vi "1g_v4.vi"() -> ()   [LabVIEW 2017]
uses:
  <vilib>/Instr/_visa.llb/VISA Configure Serial Port (Instr).vi
panel:
  in  "stop":bool
  out "Spectrometer Information":string
  out "Spectrometer Name":string
  in  "Integration Time 100 tp 250 milliseconds":dbl=100.0 min=100.0 max=500.0 step=50.0
  out "XY Graph":cluster{dbl[], u16[]}(graph)
  out "VISA resource name out":refnum<visa-resource-name>
  in  "VISA resource name":refnum<visa-resource-name>="COM3" caption="Serial COM port"
  # "REAL TIME FIBER OPTIC TEMPERATURE MONITORING SYSTEM"
  # "Partially working code"
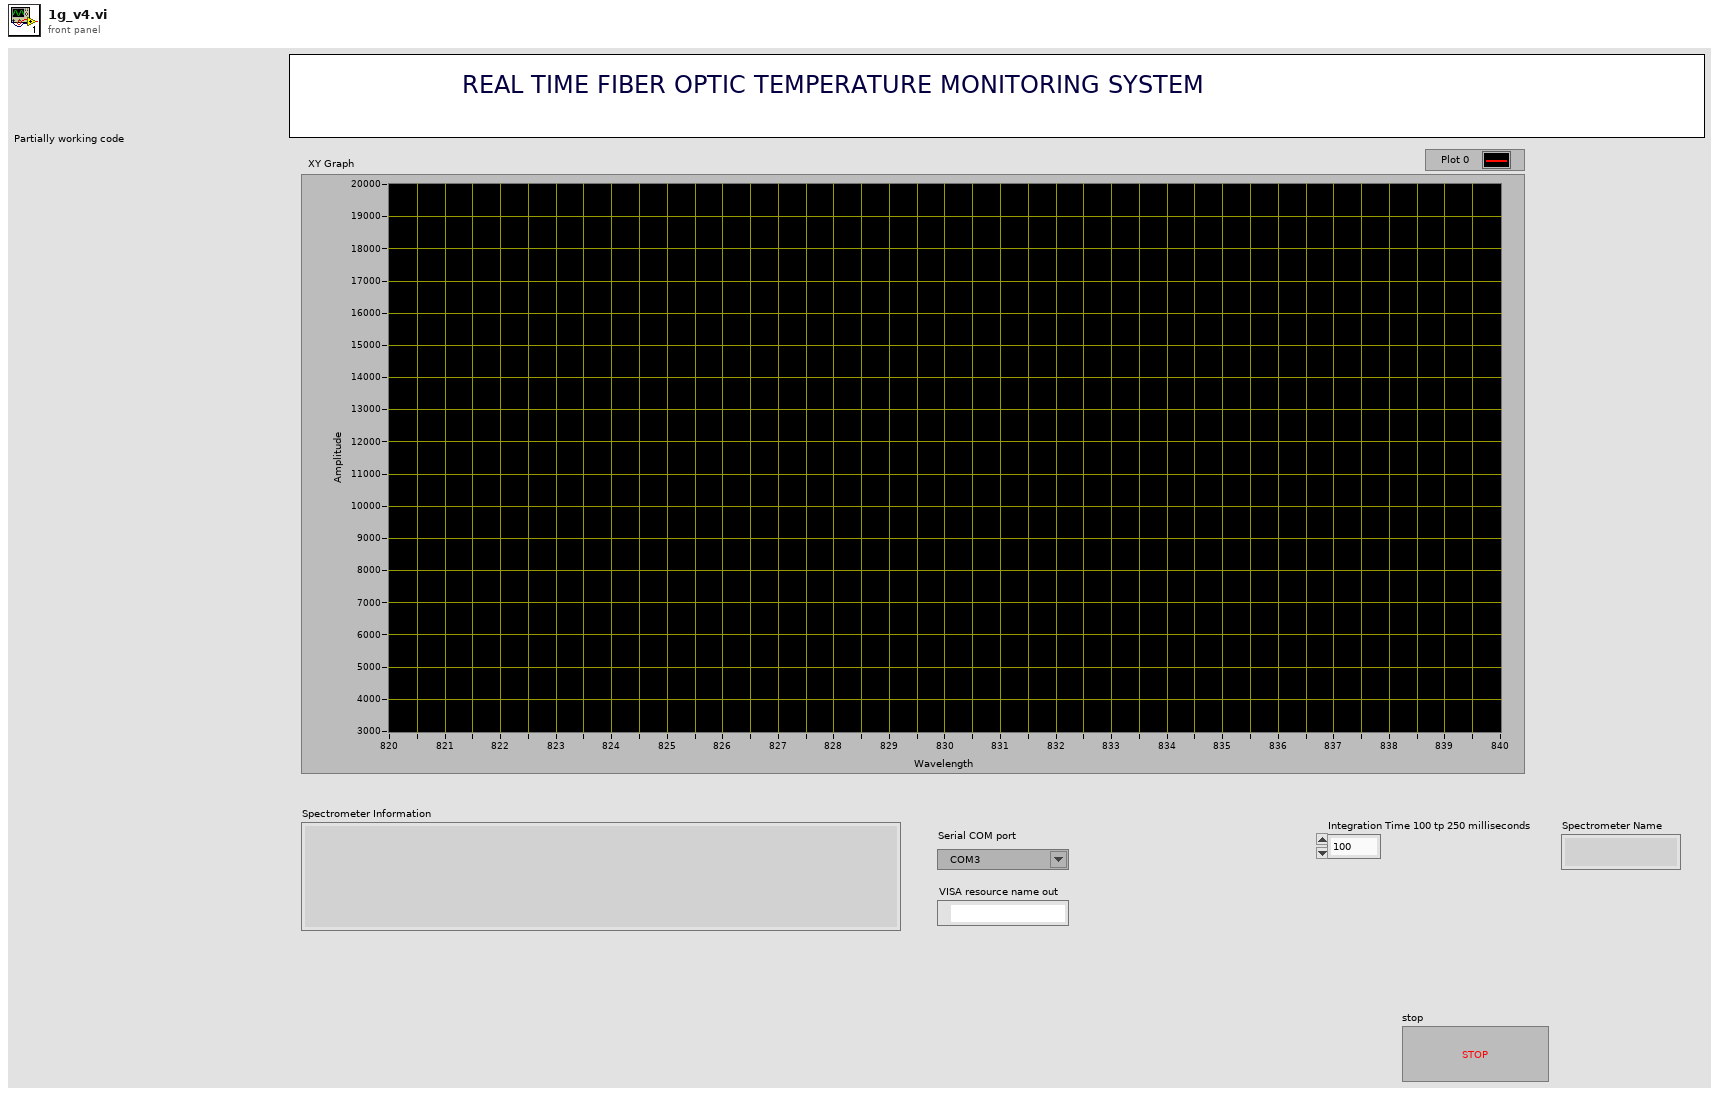
[diagram p1: front panel]
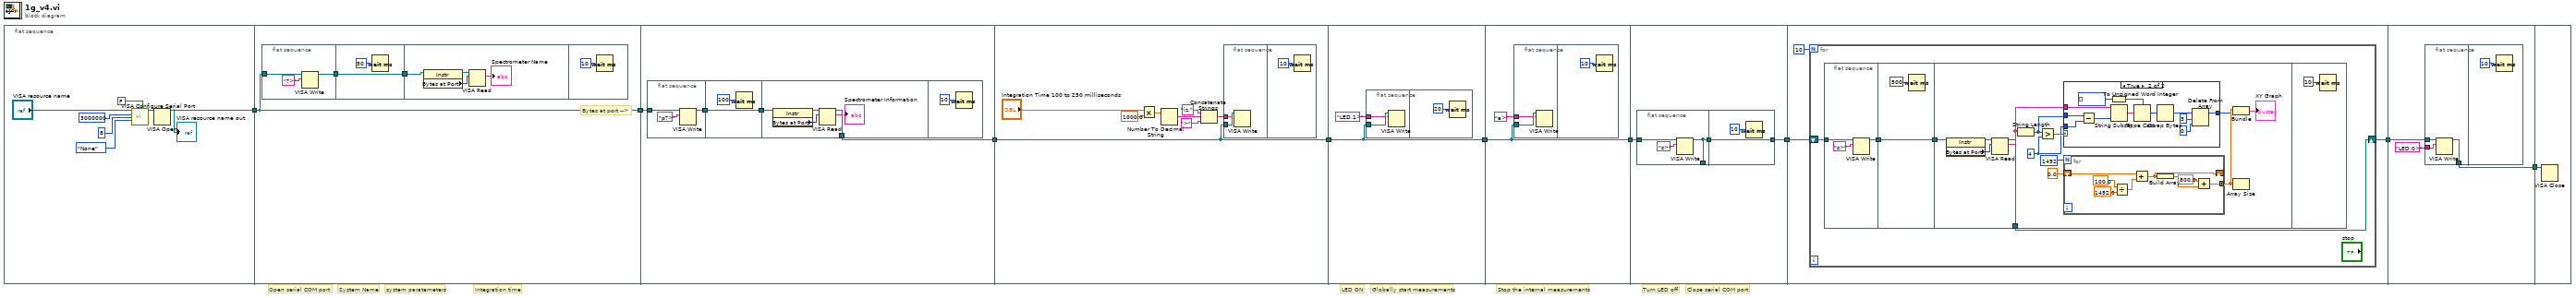
[diagram p0: block diagram]
diagram:
  # "Globally start measurements"
  # "LED ON"
  # "System Name"
  # "Integration time"
  # "system paratemeters"
  # "Close serial COM port"
  # "Turn LED off"
  # "Stop the internal measurements"
  # "Open serial COM port"
  n1 = flat-sequence {
    tunnel: [w10] -> w3
    tunnel: [w17] -> w9
    tunnel: w3 -> [w17]
    tunnel: w9 -> [w31]
    tunnel: [w30] -> w8
    tunnel: w8 -> [w48]
    tunnel: [w48] -> w7
    tunnel: w7 -> [w56]
    tunnel: [w56] -> w4
    tunnel: [w61] -> w2
    tunnel: w4 -> [w61]
    tunnel: w2 -> [w68]
    tunnel: [w66] -> w1
    tunnel: [w76] -> w6
    tunnel: w1 -> [w75]
    tunnel: w6 -> [w121]
    tunnel: [w120] -> w5
    tunnel: w5 -> [w127]
    frame #0 {
      n2 = call-poly "VISA Configure Serial Port"("VISA resource name"="VISA resource name", "Enable Termination\nChar (T)"=FALSE ("Enable Termination\nChar (T)"), "baud rate (9600)"=u32 3000000, "data bits (8)"=u16 8, "parity (0:none)"=enum16{"None", "Odd", "Even", "Mark", "Space"}."None") -> ("VISA resource name out"=w16:refnum<visa-resource-name>)  [unwired: 9 in, 1 out]
      n3 = VISA Open(VISA resource name=w16) -> (VISA resource name=w10:refnum<visa-resource-name>)  [unwired: 4 in, 1 out]
      "VISA resource name out" <- w10
    }
    frame #1 {
      # "Bytes at port -->"
      n4 = flat-sequence {
        tunnel: [w22] -> w19
        tunnel: w17 -> [w21]
        tunnel: [w23] -> w18
        tunnel: w19 -> [w23]
        tunnel: w18 -> [w28]
        frame #0 {
          n5 = VISA Write(VISA resource name=w21, write buffer="?>") -> (VISA resource name out=w22:refnum<visa-resource-name>)  [unwired: 1 in, 2 out]
        }
        frame #1 {
          n6 = Wait (ms)(milliseconds to wait=u32 50 ("Zu wartende ms")) -> ()  [unwired: 1 out]
        }
        frame #2 {
          n7 = property class="Instr"(reference=w28) -> (reference out=w27:refnum<visa-resource-name>, "Bytes at Port"=w26:u32)  [unwired: 1 in, 1 out]
          n8 = VISA Read(VISA resource name=w27, byte count=w26) -> (read buffer=→"Spectrometer Name":string)  [unwired: 1 in, 3 out]
        }
        frame #3 {
          n9 = Wait (ms)(milliseconds to wait=u32 10 ("Zu wartende ms")) -> ()  [unwired: 1 out]
        }
      }
    }
    frame #2 {
      n10 = flat-sequence {
        tunnel: [w36] -> w33
        tunnel: w31 -> [w34]
        tunnel: [w37] -> w32
        tunnel: w33 -> [w37]
        tunnel: w32 -> [w43]
        tunnel: [w40] -> w30
        frame #0 {
          n11 = VISA Write(VISA resource name=w34, write buffer="p?>") -> (VISA resource name out=w36:refnum<visa-resource-name>)  [unwired: 1 in, 2 out]
        }
        frame #1 {
          n12 = Wait (ms)(milliseconds to wait=u32 100 ("Zu wartende ms")) -> ()  [unwired: 1 out]
        }
        frame #2 {
          n13 = property class="Instr"(reference=w43) -> (reference out=w42:refnum<visa-resource-name>, "Bytes at Port"=w41:u32)  [unwired: 1 in, 1 out]
          n14 = VISA Read(VISA resource name=w42, byte count=w41) -> (VISA resource name out=w40:refnum<visa-resource-name>, read buffer=→"Spectrometer Information":string)  [unwired: 1 in, 2 out]
        }
        frame #3 {
          n15 = Wait (ms)(milliseconds to wait=u32 10 ("Zu wartende ms")) -> ()  [unwired: 1 out]
        }
      }
    }
    frame #3 {
      n16 = Multiply(x="Integration Time 100 tp 250 milliseconds", y=1000.0) -> (x*y=w45:dbl)
      n17 = Number To Decimal String(number=w45) -> (decimal integer string=w52:string)  [unwired: 1 in]
      n18 = Concatenate Strings("iz," ("String"), w52, ">" ("String")) -> (w49:string)
      n19 = flat-sequence {
        tunnel: w48 -> [w54]
        tunnel: w49 -> [w53]
        frame #0 {
          n20 = VISA Write(VISA resource name=w54, write buffer=w53) -> ()  [unwired: 1 in, 3 out]
        }
        frame #1 {
          n21 = Wait (ms)(milliseconds to wait=u32 10 ("Zu wartende ms")) -> ()  [unwired: 1 out]
        }
      }
    }
    frame #4 {
      n22 = flat-sequence {
        tunnel: w56 -> [w59]
        tunnel: "LED,1>" ("String") -> [w58]
        frame #0 {
          n23 = VISA Write(VISA resource name=w59, write buffer=w58) -> ()  [unwired: 1 in, 3 out]
        }
        frame #1 {
          n24 = Wait (ms)(milliseconds to wait=u32 20 ("Zu wartende ms")) -> ()  [unwired: 1 out]
        }
      }
    }
    frame #5 {
      n25 = flat-sequence {
        tunnel: w61 -> [w64]
        tunnel: "a>" ("String") -> [w63]
        frame #0 {
          n26 = VISA Write(VISA resource name=w64, write buffer=w63) -> ()  [unwired: 1 in, 3 out]
        }
        frame #1 {
          n27 = Wait (ms)(milliseconds to wait=u32 10 ("Zu wartende ms")) -> ()  [unwired: 1 out]
        }
      }
    }
    frame #6 {
      n28 = flat-sequence {
        tunnel: [w69] -> _
        tunnel: w68 -> [w70]
        tunnel: [w69] -> w67
        tunnel: [w73] -> w66
        tunnel: w67 -> [w73]
        frame #0 {
          n29 = VISA Write(VISA resource name=w70, write buffer="s>") -> (VISA resource name out=w69:refnum<visa-resource-name>)  [unwired: 1 in, 2 out]
        }
        frame #1 {
          n30 = Wait (ms)(milliseconds to wait=u32 10) -> ()  [unwired: 1 out]
        }
      }
    }
    frame #7 {
      n31 = for {
        N: 10 -> [_]
        shift-right: [w78] -> w76
        shift-left: w75 -> [w77]
        n32 = flat-sequence {
          tunnel: [w83] -> w80
          tunnel: w77 -> [w81]
          tunnel: [w84] -> w79
          tunnel: w80 -> [w84]
          tunnel: w79 -> [w93]
          tunnel: [w92] -> w78
          frame #0 {
            n33 = VISA Write(VISA resource name=w81, write buffer="s>") -> (VISA resource name out=w83:refnum<visa-resource-name>)  [unwired: 1 in, 2 out]
          }
          frame #1 {
            n34 = Wait (ms)(milliseconds to wait=u32 500 ("Zu wartende ms")) -> ()  [unwired: 1 out]
          }
          frame #2 {
            w86 = 4 ("y")
            n35 = property class="Instr"(reference=w93) -> (reference out=w91:refnum<visa-resource-name>, "Bytes at Port"=w90:u32)  [unwired: 1 in, 1 out]
            n36 = VISA Read(VISA resource name=w91, byte count=w90) -> (VISA resource name out=w92:refnum<visa-resource-name>, read buffer=w89:string)  [unwired: 1 in, 2 out]
            n37 = String Length(string=w89) -> (length=w88:i32)
            n38 = Greater?(x=w88, y=w86) -> (0:w87:bool)
            n39 = case shown="True" w87 {
              tunnel: w89 -> [_ w110]
              tunnel: w88 -> [_ w109]
              tunnel: w86 -> [_ w108]
              tunnel: [_ w99] -> w96
              frame False {
              }
              frame True {
                n40 = Subtract(x=w109, y=w108) -> (x-y=w107:i32)
                n41 = To Unsigned Word Integer(number=i32[] []) -> (unsigned 16bit integer=w106:u16[])
                n42 = String Subset(string=w110, length (rest)=w107) -> (substring=w105:string)  [unwired: 1 in]
                n43 = Type Cast(type=w106, x=w105) -> (*(type *) &x=w103:u16[])
                n44 = Swap Bytes(anything=w103) -> (byte swapped=w102:u16[])
                n45 = Delete From Array(array=w102, length=3, index=0) -> (array with subset deleted=w99:u16[])  [unwired: 1 out]
              }
            }
            n46 = for {
              N: 1492 -> [_]
              shift-right: [w117] -> _
              shift-left: 0.0 -> [w118]
              tunnel: [w114] -> w98 mode=concatenating
              n47 = Divide(x=100.0 ("x/y"), y=1492.0) -> (x/y=w111:dbl)
              n48 = Add(x=w118, y=w111) -> (x+y=w117:dbl)
              n49 = Build Array(w117) -> (w115:dbl[])
              n50 = Add(x=800.0 ("x+y"), y=w115) -> (x+y=w114:dbl[])
            }
            n51 = Bundle(w98, w96) -> (→"XY Graph":cluster{dbl[], u16[]})  [unwired: 1 in]
            n52 = Array Size(array=w98) -> ()  [unwired: 1 out]
          }
          frame #3 {
            n53 = Wait (ms)(milliseconds to wait=u32 10 ("Zu wartende ms")) -> ()  [unwired: 1 out]
          }
        }
      }
    }
    frame #8 {
      n54 = flat-sequence {
        tunnel: w121 -> [w125]
        tunnel: "LED,0>" ("String") -> [w124]
        tunnel: [w123] -> w120
        frame #0 {
          n55 = VISA Write(VISA resource name=w125, write buffer=w124) -> (VISA resource name out=w123:refnum<visa-resource-name>)  [unwired: 1 in, 2 out]
        }
        frame #1 {
          n56 = Wait (ms)(milliseconds to wait=u32 10 ("Zu wartende ms")) -> ()  [unwired: 1 out]
        }
      }
    }
    frame #9 {
      n57 = VISA Close(VISA resource name=w127) -> ()  [unwired: 1 in, 1 out]
    }
  }
